vi "Test_Draw.vi"(11 "Rows":i32[](array[numeric])=[7, 7, 8, 6, 7]) -> ()   [LabVIEW 2026]
doc: "UI_Draw_Board 테스트: 정수 배열로 돌을 놓고 Picture에 그린다."
panel:
  out "error out":errorcluster
  in  "PNG Path":path
  in  "Win Line From First 5":bool
  in  "Hover Col":i32=9
  in  "Hover Row":i32=9
  in  "Stones":i32[](array[numeric])=[1, 2, 1, 2, 1]
  in  "Cols":i32[](array[numeric])=[7, 8, 7, 6, 9]
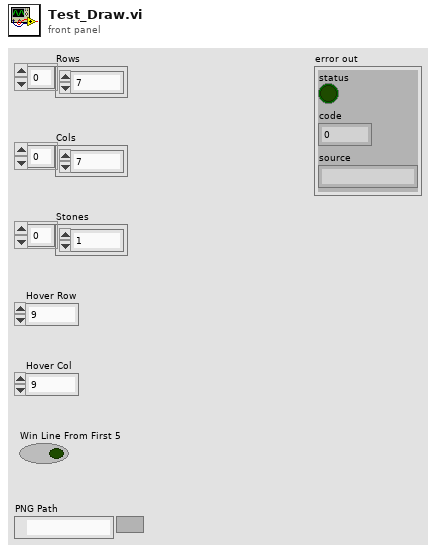
[diagram p1: front panel]
types:
  T1 = cluster{"left":i16, "top":i16, "right":i16, "bottom":i16}
  T2 = cluster{"Row":i32, "Col":i32, "Stone":enum8{"Empty", "Black", "White"}}[]
  T3 = cluster{"Row":i32, "Col":i32, "Stone":enum8{"Empty", "Black", "White"}}
  T4 = cluster{"Grid":enum8{"Empty", "Black", "White"}[][], "Move History":cluster{"Row":i32, "Col":i32, "Stone":enum8{"Empty", "Black", "White"}}[], "Last Move":cluster{"Row":i32, "Col":i32, "Stone":enum8{"Empty", "Black", "White"}}}
  T5 = typedef "imagedata.ctl" = cluster{"image type":i32, "image depth":i32, "image":u8[], "mask":u8[], "colors":u32[], "Rectangle":cluster{"left":i16, "top":i16, "right":i16, "bottom":i16}}
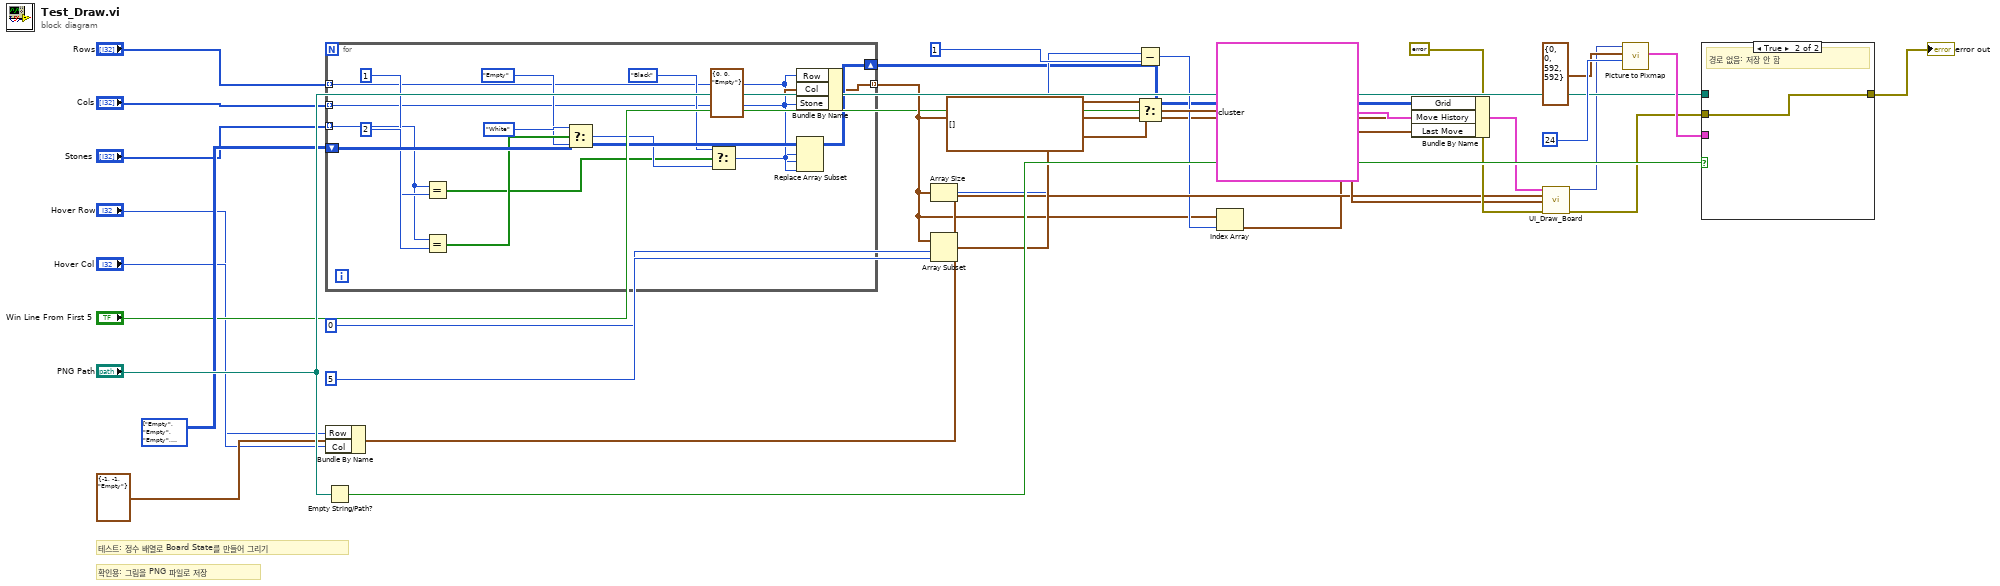
[diagram p0: block diagram]
diagram:
  w7 = enum8{"Empty", "Black", "White"}[][] [[enum."Empty", enum."Empty", enum."Empty", enum."Empty", enum."Empty", enum."Empty", enum."Empty", enum."Empty", enum."Empty", enum."Empty", enum."Empty", enum."Empty", enum."Empty", enum."Empty", enum."Empty"], [enum."Empty", enum."Empty", enum."Empty", enum."Empty", enum."Empty", enum."Empty", enum."Empty", enum."Empty", enum."Empty", enum."Empty", enum."Empty", enum."Empty", enum."Empty", enum."Empty", enum."Empty"], [enum."Empty", enum."Empty", enum."Empty", enum."Empty", enum."Empty", enum."Empty", enum."Empty", enum."Empty", enum."Empty", enum."Empty", enum."Empty", enum."Empty", enum."Empty", enum."Empty", enum."Empty"], [enum."Empty", enum."Empty", enum."Empty", enum."Empty", enum."Empty", enum."Empty", enum."Empty", enum."Empty", enum."Empty", enum."Empty", enum."Empty", enum."Empty", enum."Empty", enum."Empty", enum."Empty"], [enum."Empty", enum."Empty", enum."Empty", enum."Empty", enum."Empty", enum."Empty", enum."Empty", enum."Empty", enum."Empty", enum."Empty", enum."Empty", enum."Empty", enum."Empty", enum."Empty", enum."Empty"], [enum."Empty", enum."Empty", enum."Empty", enum."Empty", enum."Empty", enum."Empty", enum."Empty", enum."Empty", enum."Empty", enum."Empty", enum."Empty", enum."Empty", enum."Empty", enum."Empty", enum."Empty"], [enum."Empty", enum."Empty", enum."Empty", enum."Empty", enum."Empty", enum."Empty", enum."Empty", enum."Empty", enum."Empty", enum."Empty", enum."Empty", enum."Empty", enum."Empty", enum."Empty", enum."Empty"], [enum."Empty", enum."Empty", enum."Empty", enum."Empty", enum."Empty", enum."Empty", enum."Empty", enum."Empty", enum."Empty", enum."Empty", enum."Empty", enum."Empty", enum."Empty", enum."Empty", enum."Empty"], [enum."Empty", enum."Empty", enum."Empty", enum."Empty", enum."Empty", enum."Empty", enum."Empty", enum."Empty", enum."Empty", enum."Empty", enum."Empty", enum."Empty", enum."Empty", enum."Empty", enum."Empty"], [enum."Empty", enum."Empty", enum."Empty", enum."Empty", enum."Empty", enum."Empty", enum."Empty", enum."Empty", enum."Empty", enum."Empty", enum."Empty", enum."Empty", enum."Empty", enum."Empty", enum."Empty"], [enum."Empty", enum."Empty", enum."Empty", enum."Empty", enum."Empty", enum."Empty", enum."Empty", enum."Empty", enum."Empty", enum."Empty", enum."Empty", enum."Empty", enum."Empty", enum."Empty", enum."Empty"], [enum."Empty", enum."Empty", enum."Empty", enum."Empty", enum."Empty", enum."Empty", enum."Empty", enum."Empty", enum."Empty", enum."Empty", enum."Empty", enum."Empty", enum."Empty", enum."Empty", enum."Empty"], [enum."Empty", enum."Empty", enum."Empty", enum."Empty", enum."Empty", enum."Empty", enum."Empty", enum."Empty", enum."Empty", enum."Empty", enum."Empty", enum."Empty", enum."Empty", enum."Empty", enum."Empty"], [enum."Empty", enum."Empty", enum."Empty", enum."Empty", enum."Empty", enum."Empty", enum."Empty", enum."Empty", enum."Empty", enum."Empty", enum."Empty", enum."Empty", enum."Empty", enum."Empty", enum."Empty"], [enum."Empty", enum."Empty", enum."Empty", enum."Empty", enum."Empty", enum."Empty", enum."Empty", enum."Empty", enum."Empty", enum."Empty", enum."Empty", enum."Empty", enum."Empty", enum."Empty", enum."Empty"]] items=["Empty", "Black", "White"]
  # "확인용: 그림을 PNG 파일로 저장"
  # "테스트: 정수 배열로 Board State를 만들어 그리기"
  n1 = for {
    tunnel: "Rows" -> [w32] mode=indexing
    tunnel: "Cols" -> [w33] mode=indexing
    tunnel: "Stones" -> [w34] mode=indexing
    shift-right: [w46] -> w9
    shift-left: w7 -> [w47]
    tunnel: [w45] -> w8 mode=indexing
    n2 = Equal?(x=w34, y=1) -> (x = y?=w39:bool[])
    n3 = Equal?(x=w34, y=2) -> (x = y?=w41:bool[])
    n4 = Select(t=enum8{"Empty", "Black", "White"}."White", s=w41, f=enum8{"Empty", "Black", "White"}."Empty") -> (s? t:f=w42:enum8{"Empty", "Black", "White"})
    n5 = Select(t=enum8{"Empty", "Black", "White"}."Black", s=w39, f=w42) -> (s? t:f=w43:enum8{"Empty", "Black", "White"})
    n6 = Bundle By Name(cluster=T3 {"Row"=0, "Col"=0, "Stone"=enum."Empty"}, "Row"=w32, "Col"=w33, "Stone"=w43) -> (w45:T3)
    n7 = Replace Array Subset(array=w47, new element=w43, index (row)=w32, index (col)=w33) -> (w46:enum8{"Empty", "Black", "White"}[][])
  }
  n8 = Bundle By Name(cluster=T3 {"Row"=-1, "Col"=-1, "Stone"=enum."Empty"}, "Row"="Hover Row", "Col"="Hover Col") -> (w17:T3)
  n9 = Empty String/Path?(string/path="PNG Path") -> (empty?=w30:bool)
  n10 = Array Size(array=w8) -> (size(s)=w10:i32)
  n11 = Array Subset(array=w8, index=0, length=5) -> (w20:T2)
  n12 = Subtract(x=w10, y=1) -> (x-y=w12:i32)
  n13 = Select(t=w20, s="Win Line From First 5", f=T2 []) -> (s? t:f=w22:T2)
  n14 = Index Array(array=w8, index=w12) -> (element=w13:T3)
  n15 = Bundle By Name(cluster=T4 {"Grid"=array15x15[225 elements], "Move History"=[], "Last Move"={"Row"=-1, "Col"=-1, "Stone"=enum."Empty"}}, "Grid"=w9, "Move History"=w8, "Last Move"=w13) -> (w15:T4)
  n16 = call "UI_Draw_Board.vi"("Board State"=w15, "Hover"=w17, "Win Line"=w22, "error in"=errorcluster {"status"=FALSE, "code"=0, "source"=""}) -> ("Picture"=w24:picture, "error out"=w25:errorcluster)  [unwired: 10 in]
  n17 = call <vilib>:"Picture to Pixmap.vi"("depth"=24, "rect"=T1 {"left"=0, "top"=0, "right"=592, "bottom"=592}, "picture"=w24) -> ("image data"=w29:T5)  [unwired: 7 in, 1 out]
  n18 = case shown="True" w30 {
    tunnel: "PNG Path" -> [w49 _]
    tunnel: w25 -> [w48 w52]
    tunnel: w29 -> [w50 _]
    tunnel: [w51 w52] -> w31
    frame False {
      # "PNG 저장"
      n19 = call <vilib>:"Write PNG File.vi"("error in (no error)"=w48, "image data"=w50, "path to PNG file"=w49) -> ("error out"=w51:errorcluster)  [unwired: 7 in, 1 out]
    }
    frame True {
      # "경로 없음: 저장 안 함"
    }
  }
  "error out" <- w31
